vi "表格组合事件.vi"(4 "颜色":u32(colorbox)=6618880, 6 "类型":enum16{"无", "单格", "整行", "整列"}(ring)=enum."单格", 9 "字符串":string, 10 "Row":i32, 11 "Col":i32) -> (2 "结果字符串":string)   [LabVIEW 2025]
uses:
  global.vi
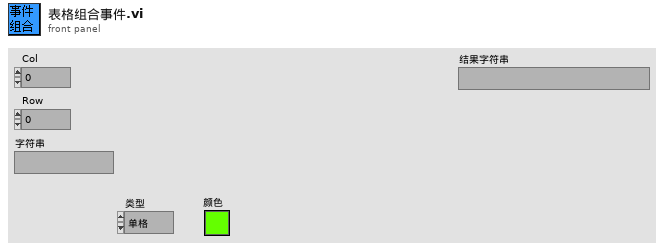
[diagram p1: front panel]
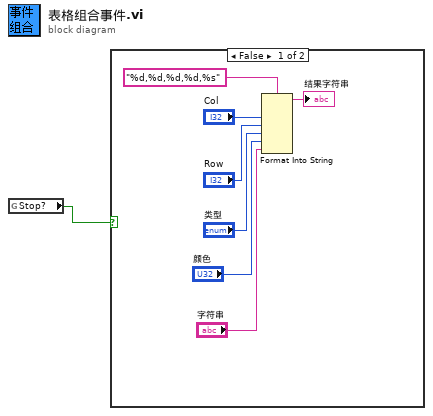
[diagram p0: block diagram]
diagram:
  n1 = global read "global.vi" "Stop?"() -> (w1:bool)
  n2 = case shown="False" w1 {
    frame False {
      n3 = Format Into String(format string="%d,%d,%d,%d,%s" ("格式字符串"), "Col", "Row", "类型", "颜色", "字符串") -> (resulting string=→"结果字符串":string)  [unwired: 2 in, 1 out]
    }
    frame True {
    }
  }
